vi "test_InitializeItemContents.vi"() -> (2 "Actuals":T1[](array[typedef]), 3 "Pass?":bool)   [LabVIEW 2020, in "Tests.LabVIEWItem.lvlib"]
uses:
  Tests.LabVIEWItem.lvlib
  Validation/Validate_BaseConstruction.ctl
  CLabVIEWItem/CLabVIEWItem.lvclass
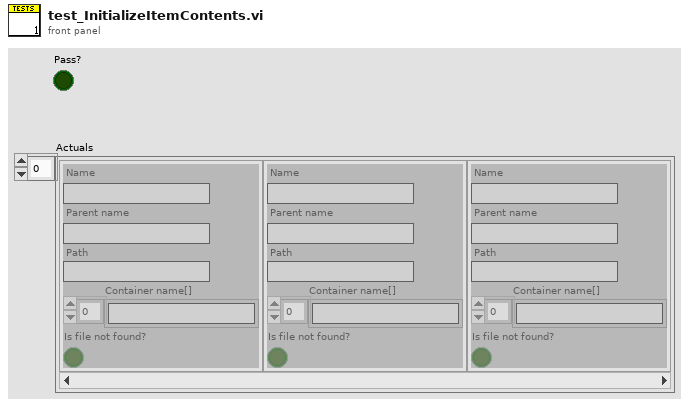
[diagram p1: front panel]
types:
  T1 = typedef "Tests.LabVIEWItem.lvlib/Validate_BaseConstruction.ctl" = cluster{"Name":string, "Parent name":string, "Path":string, "Container name[]":string[], "Is file not found?":bool}
  T2 = typedef "Tests.LabVIEWItem.lvlib/Params_ConstructLabVIEWItem.ctl" = cluster{"Input":T3, "Validation":T1}
  T3 = typedef "Tests.LabVIEWItem.lvlib/Input_BaseConstruction.ctl" = cluster{"Qualified name":string, "Path":string, "Error code":i32}
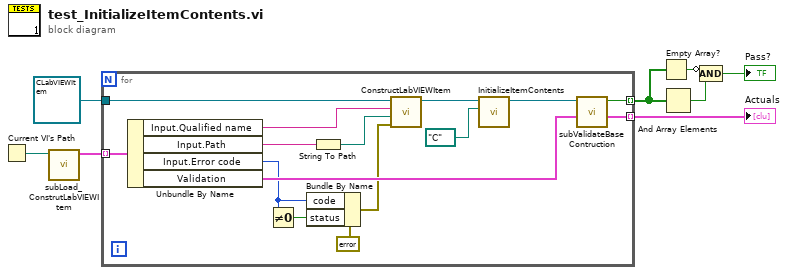
[diagram p0: block diagram]
diagram:
  n1 = Current VI's Path() -> (path=w7:path)
  n2 = call "subLoad_ConstrutLabVIEWItem.vi"("Caller path"=w7) -> ("Params"=w6:T2[])  [unwired: 10 in]
  n3 = for {
    tunnel: refnum<class "CLabVIEWItem.lvclass"> refnum ("CLabVIEWItem in") -> [w23]
    tunnel: [w22] -> w1 mode=indexing
    tunnel: w6 -> [w20] mode=indexing
    tunnel: [w21] -> w5 mode=indexing
    n4 = Unbundle By Name(w20) -> ("Input.Qualified name"=w18:string, "Input.Path"=w17:string, "Input.Error code"=w13:i32, "Validation"=w19:T1)
    n5 = Not Equal To 0?(x=w13) -> (x != 0?=w12:bool)
    n6 = Bundle By Name(cluster=errorcluster {"status"=FALSE, "code"=0, "source"=""} ("error in (no error)"), "code"=w13, "status"=w12) -> (w14:errorcluster)
    n7 = String To Path(string=w17) -> (path=w16:path)
    n8 = call-dynamic "ConstructLabVIEWItem.vi"("error in (no error)"=w14, "Path"=w16, "Qualified name"=w18, "CLabVIEWItem in"=w23) -> ("CLabVIEWItem out"=w11:refnum<class "CLabVIEWItem.lvclass">)  [unwired: 6 in, 1 out]
    n9 = call-dynamic "InitializeItemContents.vi"("Root path"=path "C:/", "CLabVIEWItem in"=w11) -> ("CLabVIEWItem out"=w10:refnum<class "CLabVIEWItem.lvclass">)  [unwired: 8 in, 1 out]
    n10 = call "subValidateBaseContruction.vi"("Parameters"=w19, "CLabVIEWItem in"=w10) -> ("Actual"=w22:T1, "Pass?"=w21:bool)  [unwired: 8 in]
  }
  "Actuals" <- w1
  n11 = Empty Array?(array=w5) -> (empty?=w4:bool)
  n12 = And Array Elements(Boolean array=w5) -> (logical AND=w3:bool)
  n13 = Compound Arithmetic op=AND(invert w4, w3) -> (→"Pass?":bool)
